vi "Read Variant OPC.vi"(8 "error in (no error)":errorcluster, 10 "data":variant, 11 "URL":string) -> (0 "error out":errorcluster, 3 "Desc":string)   [LabVIEW 2012]
uses:
  write_String.vi
  write_Num.vi
  write_bool.vi
  write_Array.vi
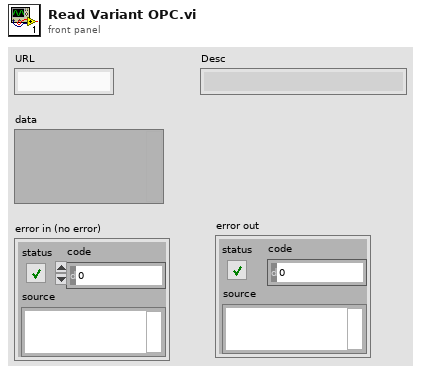
[diagram p1: front panel]
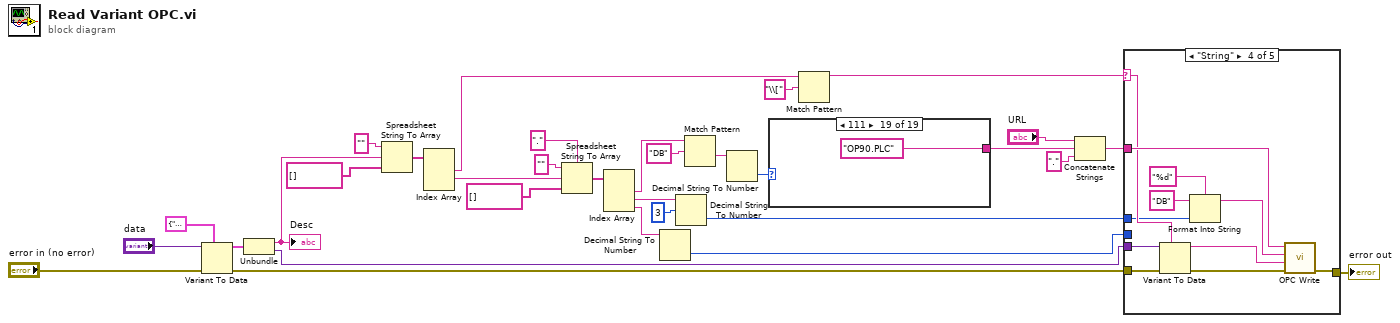
[diagram p0: block diagram]
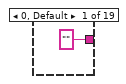
[diagram p2: hidden frame]
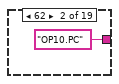
[diagram p3: hidden frame]
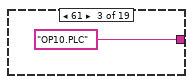
[diagram p4: hidden frame]
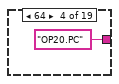
[diagram p5: hidden frame]
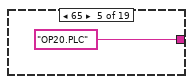
[diagram p6: hidden frame]
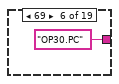
[diagram p7: hidden frame]
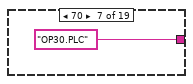
[diagram p8: hidden frame]
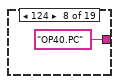
[diagram p9: hidden frame]
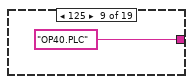
[diagram p10: hidden frame]
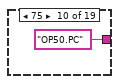
[diagram p11: hidden frame]
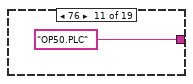
[diagram p12: hidden frame]
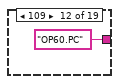
[diagram p13: hidden frame]
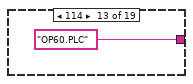
[diagram p14: hidden frame]
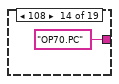
[diagram p15: hidden frame]
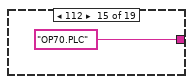
[diagram p16: hidden frame]
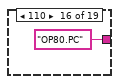
[diagram p17: hidden frame]
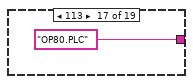
[diagram p18: hidden frame]
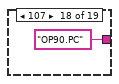
[diagram p19: hidden frame]
diagram:
  n1 = Variant To Data(error in="error in (no error)", type=cluster{"Desc":string, "NewVal":variant} {"Desc"="", "NewVal"=variant} ("output cluster"), Variant="data") -> (data=w24:cluster{"Desc":string, "NewVal":variant}, error out=w31:errorcluster)
  n2 = Unbundle(w24) -> ("Desc"=w26:string, "NewVal"=w29:variant)
  "Desc" <- w26
  n3 = Spreadsheet String To Array(format string="", spreadsheet string=w26, array type (2D Dbl)=string[] [] ("Device ID")) -> (array=w28:string[])  [unwired: 1 in]
  n4 = Index Array(array=w28) -> (element #1=w16:string, element #2=w20:string)  [unwired: 3 in, 1 out]
  n5 = Spreadsheet String To Array(delimiter (Tab)=".", format string="", spreadsheet string=w20, array type (2D Dbl)=string[] [] ("Device ID")) -> (array=w18:string[])
  n6 = Index Array(array=w18) -> (element #1=w11:string, element #2=w13:string, element #3=w17:string)  [unwired: 3 in]
  n7 = Decimal String To Number(string=w17) -> (number=w3:i32)  [unwired: 2 in, 1 out]
  n8 = Decimal String To Number(string=w13, offset=3) -> (number=w4:i32)  [unwired: 1 in, 1 out]
  n9 = Match Pattern(string=w11, regular expression="DB") -> (after substring=w9:string)  [unwired: 1 in, 3 out]
  n10 = Decimal String To Number(string=w9) -> (number=w8:i32)  [unwired: 2 in, 1 out]
  n11 = case shown="111" w8 {
    tunnel: ["" ("URL") "OP10.PC" ("URL") "OP10.PLC" ("URL") "OP20.PC" ("URL") "OP20.PLC" ("URL") "OP30.PC" ("URL") "OP30.PLC" ("URL") "OP40.PC" ("URL") "OP40.PLC" ("URL") "OP50.PC" ("URL") "OP50.PLC" ("URL") "OP60.PC" ("URL") "OP60.PLC" ("URL") "OP70.PC" ("URL") "OP70.PLC" ("URL") "OP80.PC" ("URL") "OP80.PLC" ("URL") "OP90.PC" ("URL") "OP90.PLC" ("URL")] -> w6
    frame 0, Default {
    }
    frame 62 {
    }
    frame 61 {
    }
    frame 64 {
    }
    frame 65 {
    }
    frame 69 {
    }
    frame 70 {
    }
    frame 124 {
    }
    frame 125 {
    }
    frame 75 {
    }
    frame 76 {
    }
    frame 109 {
    }
    frame 114 {
    }
    frame 108 {
    }
    frame 112 {
    }
    frame 110 {
    }
    frame 113 {
    }
    frame 107 {
    }
    frame 111 {
    }
  }
  n12 = Match Pattern(string=w16, regular expression="\\[") -> (before substring=w14:string)  [unwired: 1 in, 3 out]
  n13 = Concatenate Strings("URL", w6, "." ("string")) -> (w5:string)
  n14 = case shown="\"String\"" w14 {
    selector: w14 -> [_ _ _ w84 _]
    tunnel: w5 -> [_ w64 w74 w85 w95]
    tunnel: w29 -> [_ w63 w71 w83 w94]
    tunnel: w31 -> [w52 w62 w73 w82 w93]
    tunnel: w4 -> [_ w55 w67 w77 w88]
    tunnel: w3 -> [_ w54 _ _ _]
    tunnel: [w52 w53 w65 w75 w86] -> w1
    frame Default {
    }
    frame "Bool" {
      n15 = Variant To Data(error in=w62, type=FALSE, Variant=w63) -> (data=w60:bool, error out=w59:errorcluster)
      n16 = Format Into String(format string="%d_%d", initial string="DB", w55, w54) -> (resulting string=w56:string)  [unwired: 1 in, 1 out]
      n17 = call-poly "OPC Write.vi"("错误输入（无错误）"=w59, "Value"=w60, "Address"=w56, "URL"=w64) -> ("error out"=w53:errorcluster)  [unwired: 6 in, 1 out]
    }
    frame "DInt", "Int" {
      n18 = Variant To Data(error in=w73, type=u32 50 ("milliseconds to wait"), Variant=w71) -> (data=w70:u32)  [unwired: 1 out]
      n19 = Format Into String(format string="%d", initial string="DB", w67) -> (resulting string=w66:string)  [unwired: 1 in, 1 out]
      n20 = call-poly "OPC Write.vi"("Value"=w70, "Address"=w66, "URL"=w74) -> ("error out"=w65:errorcluster)  [unwired: 7 in, 1 out]
    }
    frame "String" {
      n21 = Variant To Data(error in=w82, type=w84, Variant=w83) -> (data=w80:string, error out=w81:errorcluster)
      n22 = Format Into String(format string="%d", initial string="DB", w77) -> (resulting string=w76:string)  [unwired: 1 in, 1 out]
      n23 = call-poly "OPC Write.vi"("错误输入（无错误）"=w81, "Value"=w80, "Address"=w76, "URL"=w85) -> ("error out"=w75:errorcluster)  [unwired: 6 in, 1 out]
    }
    frame "Array" {
      n24 = Variant To Data(error in=w93, type=u8[] [] ("Device ID"), Variant=w94) -> (data=w91:u8[])  [unwired: 1 out]
      n25 = Format Into String(format string="%d", initial string="DB", w88) -> (resulting string=w87:string)  [unwired: 1 in, 1 out]
      n26 = call-poly "OPC Write.vi"("Value"=w91, "Address"=w87, "URL"=w95) -> ("error out"=w86:errorcluster)  [unwired: 7 in, 1 out]
    }
  }
  "error out" <- w1
